vi "MPExxx_get_stat_oper.vi"(0 "VISA session":refnum<visa-resource-name>, 1 "error in (no error)":errorcluster) -> (2 "dup VISA session":refnum<visa-resource-name>, 3 "Operational Status Register":string, 4 "error out":errorcluster)   [LabVIEW 2012]
doc: "This query returns the value of the Operation Register which is a read-only register that holds the real-time (un-latched) condition of the operational status of the power supply. \n\nBIT DESCRIPTION\n0 - Arm\n1 - Soft Start\n2 - InterLock\n3 - Internal Control\n4 - External Control\n5 - Interface is waiting for trigger\n6 - Standby\n7 - Power\n8 - Constant Voltage\n9 - Remote Sense\n10 - Constant Current\n11 - Standby or Alarm\n12-15 Not Used"
panel:
  # "MAGNA-POWER"
  # "Electronics"
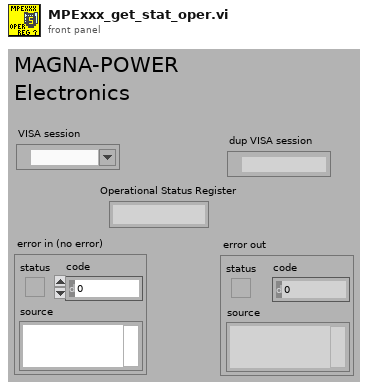
[diagram p1: front panel]
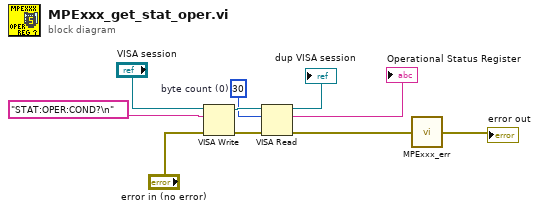
[diagram p0: block diagram]
diagram:
  w8 = u32 30  # byte count (0)
  n1 = VISA Write(VISA resource name="VISA session", write buffer="STAT:OPER:COND?\n", error in (no error)="error in (no error)") -> (VISA resource name out=w9:refnum<visa-resource-name>, error out=w7:errorcluster)  [unwired: 1 out]
  n2 = VISA Read(VISA resource name=w9, byte count=w8, error in (no error)=w7) -> (VISA resource name out=→"dup VISA session":refnum<visa-resource-name>, read buffer=→"Operational Status Register":string, error out=w2:errorcluster)  [unwired: 1 out]
  n3 = call "MPExxx_err.vi"("error in (no error)"=w2) -> ("error out"=→"error out":errorcluster)
